vi "work2_Cooker_Module.vi"() -> ()   [LabVIEW 2026]
panel:
  in  "nombre":i32
  in  "Meal":bool
  in  "stop":bool
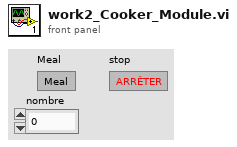
[diagram p1: front panel]
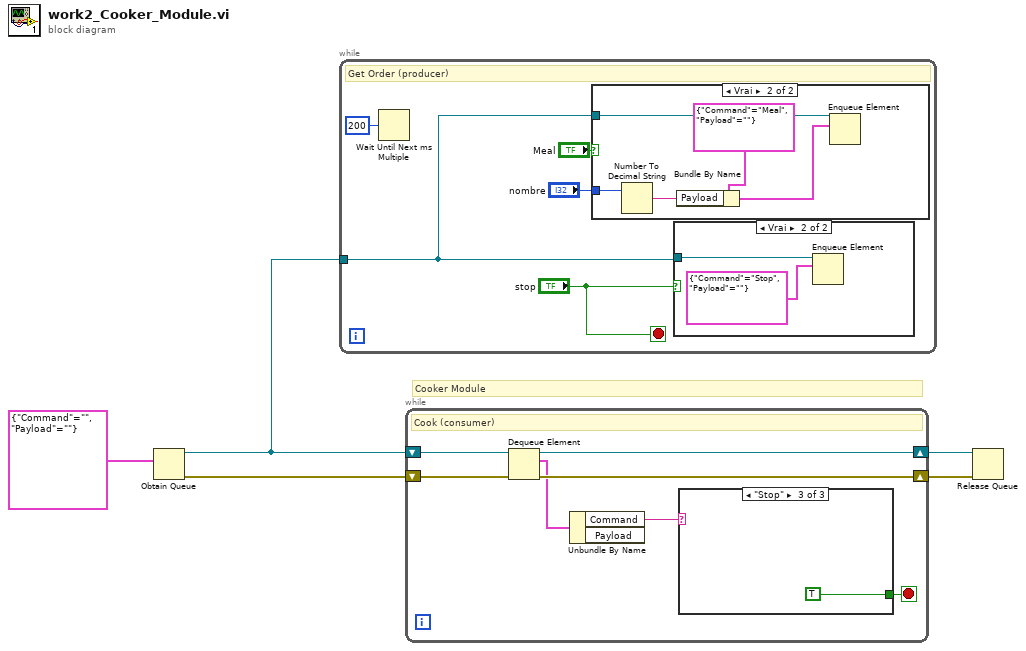
[diagram p0: block diagram]
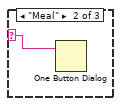
[diagram p5: hidden frame]
diagram:
  # "Cooker Module"
  n1 = Obtain Queue(element data type=cluster{"Command":string, "Payload":string} {"Command"="", "Payload"=""}) -> (queue out=w2:refnum<queue>, error out=w5:errorcluster)  [unwired: 4 in, 1 out]
  n2 = while {
    tunnel: w2 -> [w10]
    stop <- "stop" stop-if-true
    # "Get Order (producer)"
    n3 = Wait Until Next ms Multiple(millisecond multiple=u32 200 ("n millisecondes")) -> ()  [unwired: 1 out]
    n4 = case shown="Vrai" "Meal" {
      tunnel: w10 -> [_ w15]
      tunnel: "nombre" -> [_ w13]
      frame False {
      }
      frame True {
        n5 = Number To Decimal String(number=w13) -> (decimal integer string=w14:string)  [unwired: 1 in]
        n6 = Bundle By Name(cluster=cluster{"Command":string, "Payload":string} {"Command"="Meal", "Payload"=""} ("élément"), "Payload"=w14) -> (w11:cluster{"Command":string, "Payload":string})
        n7 = Enqueue Element(queue=w15, element=w11) -> ()  [unwired: 2 in, 3 out]
      }
    }
    n8 = case shown="Vrai" "stop" {
      tunnel: w10 -> [_ w17]
      frame False {
      }
      frame True {
        n9 = Enqueue Element(queue=w17, element=cluster{"Command":string, "Payload":string} {"Command"="Stop", "Payload"=""} ("élément")) -> ()  [unwired: 2 in, 3 out]
      }
    }
  }
  n10 = while {
    shift-right: [w22] -> w3
    shift-left: w5 -> [w24]
    shift-right: [w23] -> w4
    shift-left: w2 -> [w21]
    stop <- w18 stop-if-true
    # "Cook (consumer)"
    n11 = Dequeue Element(queue=w21, error in (no error)=w24) -> (queue out=w23:refnum<queue>, element=w20:cluster{"Command":string, "Payload":string}, error out=w22:errorcluster)  [unwired: 1 in, 1 out]
    n12 = Unbundle By Name(w20) -> ("Command"=w19:string)  [unwired: 1 out]
    n13 = case shown="\"Stop\"" w19 {
      selector: w19 -> [_ w25 _]
      tunnel: [_ _ TRUE] -> w18
      frame "Faux", Default {
      }
      frame "Meal" {
        n14 = One Button Dialog(message=w25) -> ()  [unwired: 1 in, 1 out]
      }
      frame "Stop" {
      }
    }
  }
  n15 = Release Queue(queue=w4, error in (no error)=w3) -> ()  [unwired: 1 in, 3 out]
